vi "Process Data.vi"(8 "error in (no error)":errorcluster, 9 "Running":refnum<vi>, 10 "XY Plot":refnum<vi>, 11 "H1FR":refnum<class "H1 Frequency Response.lvclass">) -> (0 "error out":errorcluster, 3 "H1FR out":refnum<class "H1 Frequency Response.lvclass">)   [LabVIEW 2025, in "H1 Plotter.lvlib" / "H1 Frequency Response.lvclass"]
uses:
  H1 Frequency Response.lvclass
  H1 Frequency Response.lvclass/H1 Frequency Response.ctl
  Users/Public/Documents/Sandia National Labs/TSS Plugin/Tests/XY Plotter.lvlibp/XY  Plotter/XY Plotter.lvclass
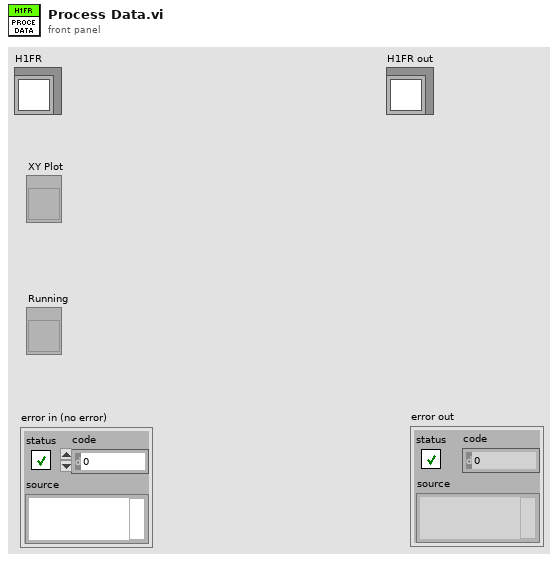
[diagram p1: front panel]
types:
  T1 = cluster{"Active Plot":u32, "XY Data":cluster{"X":dbl[], "Y":dbl[]}}
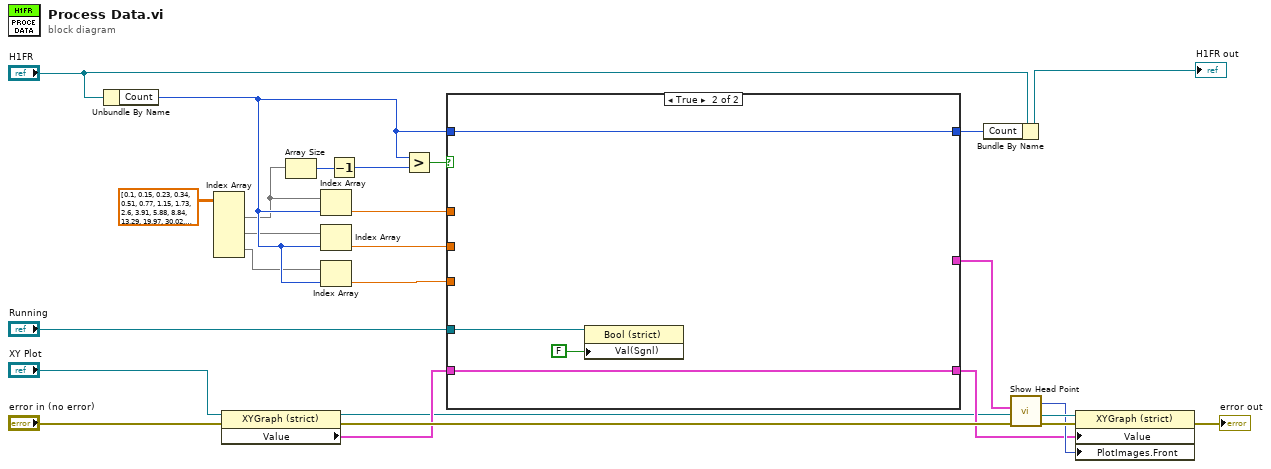
[diagram p0: block diagram]
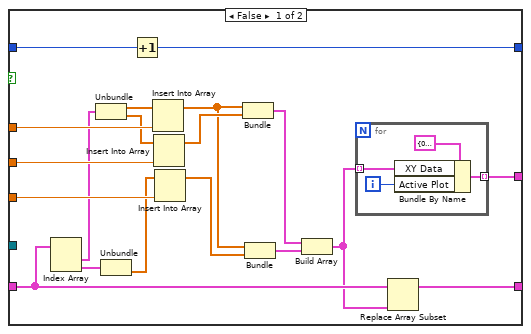
[diagram p2: hidden frame]
diagram:
  n1 = Unbundle By Name("H1FR") -> ("Count"=w21:i32)
  n2 = Index Array(array=dbl[][] [[0.1, 0.15, 0.23, 0.34, 0.51, 0.77, 1.15, 1.73, 2.6, 3.91, 5.88, 8.84, 13.29, 19.97, 30.02], [0.0, -0.01, -0.01, 0.0, 0.02, 0.0, -0.08, -0.31, -0.83, -1.96, -3.83, -6.43, -9.48, -13.24, -16.36], [1.68, 1.2, 0.49, -0.67, -2.58, -5.64, -10.01, -16.16, -24.88, -36.13, -47.67, -57.72, -63.86, -66.56, -61.68]] ("appended array")) -> (element #1=w4:dbl[], element #2=w6:dbl[], element #3=w5:dbl[])  [unwired: 6 in]
  n3 = property class="XYGraph (strict)"(reference="XY Plot", error in="error in (no error)") -> (reference out=w11:refnum<vi>, error out=w26:errorcluster, "Value"=w24:cluster{dbl[], dbl[]}[])
  n4 = Array Size(array=w4) -> (size(s)=w3:i32)
  n5 = Index Array(array=w4, index=w21) -> (element=w20:dbl)
  n6 = Index Array(array=w6, index=w21) -> (element=w19:dbl)
  n7 = Index Array(array=w5, index=w21) -> (element=w18:dbl)
  n8 = Decrement(x=w3) -> (x-1=w17:i32)
  n9 = Greater?(x=w21, y=w17) -> (0:w23:bool)
  n10 = case shown="True" w23 {
    tunnel: w21 -> [w45 w50]
    tunnel: [w44 w50] -> w25
    tunnel: "Running" -> [_ w52]
    tunnel: w20 -> [w43 _]
    tunnel: w19 -> [w42 _]
    tunnel: w18 -> [w41 _]
    tunnel: w24 -> [w30 w51]
    tunnel: [w29 w51] -> w12
    tunnel: [w27 _] -> w10
    frame False {
      n11 = Index Array(array=w30) -> (element #1=w33:cluster{dbl[], dbl[]}, element #2=w36:cluster{dbl[], dbl[]})  [unwired: 2 in]
      n12 = Unbundle(w33) -> (w32:dbl[], w31:dbl[])
      n13 = Unbundle(w36) -> (w37:dbl[])  [unwired: 1 out]
      n14 = Increment(x=w45) -> (x+1=w44:i32)
      n15 = Insert Into Array(array=w32, new element=w43) -> (w38:dbl[])  [unwired: 1 in]
      n16 = Insert Into Array(array=w31, new element=w42) -> (w39:dbl[])  [unwired: 1 in]
      n17 = Insert Into Array(array=w37, new element=w41) -> (w40:dbl[])  [unwired: 1 in]
      n18 = Bundle(w38, w39) -> (w35:cluster{dbl[], dbl[]})  [unwired: 1 in]
      n19 = Bundle(w38, w40) -> (w34:cluster{dbl[], dbl[]})  [unwired: 1 in]
      n20 = Build Array(w35, w34) -> (w28:cluster{dbl[], dbl[]}[])
      n21 = for {
        tunnel: w28 -> [w47] mode=indexing
        tunnel: [w46] -> w27 mode=indexing
        i -> [w48]
        n22 = Bundle By Name(cluster=T1 {"Active Plot"=0, "XY Data"={"X"=[], "Y"=[]}} ("Dataset"), "XY Data"=w47, "Active Plot"=w48) -> (w46:T1)
      }
      n23 = Replace Array Subset(array=w30, new element=w28) -> (w29:cluster{dbl[], dbl[]}[])  [unwired: 1 in]
    }
    frame True {
      n24 = property class="Bool (strict)"(reference=w52, "Val(Sgnl)"=FALSE ("Value (Signaling)")) -> ()  [unwired: 1 in, 2 out]
    }
  }
  n25 = Bundle By Name(cluster="H1FR", "Count"=w25) -> (→"H1FR out":refnum<class "H1 Frequency Response.lvclass">)
  n26 = call "Show Head Point.vi"("error in (no error)"=w26, "XY Plot"=w11, "DataSet"=w10) -> ("error out"=w15:errorcluster, "XY Plot out"=w14:refnum<vi>, "picture out"=w13:picture)  [unwired: 6 in]
  n27 = property class="XYGraph (strict)"(reference=w14, error in=w15, "Value"=w12, "PlotImages.Front"=w13) -> (error out=→"error out":errorcluster)  [unwired: 1 out]
